vi "RX1.vi"() -> ()   [LabVIEW 2025]
uses:
  <vilib>/addons/Modulation/Analog/support/mod_Set Error Source.vi
  <vilib>/addons/Modulation/Digital/General/MT Generate PSK System Parameters(M).vi
  <vilib>/addons/Modulation/Digital/Support/Common/Validators/mod_Generate Filter Coefficients Validate.vi
  <vilib>/addons/Modulation/Digital/General/subVIs/mod_Generate Filter Coefficients.vi
  <instrlib>/niUSRP/niUSRP Fetch Rx Data (CDB Cluster).vi
  <vilib>/addons/Modulation/niDMT.lvlib
  <vilib>/addons/Modulation/niAMT.lvlib
panel:
  in  "filter parameter":dbl=0.5 format="%.2f"
  out "Waveform Graph 3":cluster{"t0":dbl, "dt":dbl, "Y":dbl[]}(graph)
  out "hamada":errorcluster caption="error out"
  out "error out 6":errorcluster
  out "error out 4":errorcluster
  out "error out 3":errorcluster
  out "error out 2":errorcluster
  out "initiate":errorcluster
  out "output bit stream":i8[](array[numeric])
  out "Waveform Graph 2":cluster{"t0":dbl, "dt":dbl, "Y":dbl[]}(graph)
  out "measurements":T1 {"phase offset (deg)" format="%.2f"; "frequency drift (Hz)" format="%.2f"; "frequency offset (Hz)" format="%.2f"}
  out "IQ Graph":cluster{dbl[], dbl[]} {"?" format="%.2f"; "?" format="%.2f"}
  out "final error out":errorcluster
  in  "active antenna":string="RX2"
  in  "stop":bool
  in  "filter length (symbols)":i32=8
  in  "error in (no error)":errorcluster
  in  "matched samples per symbol (16)":i32=16
  in  "pulse shaping samples per symbol (16)":i32=16
  in  "differential PSK":enum16{"disable", "enable"}(ring)
  in  "M-PSK (4)":i32=8
  in  "samples per symbol (16)":i32=16
  in  "number of samples":i64=1000
  in  "gain":dbl format="%#_6f"
  in  "carrier frequency":dbl=2400000000.0 format="%#_6p"
  in  "IQ rate":dbl=200000.0 format="%#_6p"
  in  "device names":refnum<k15>="NI2900"
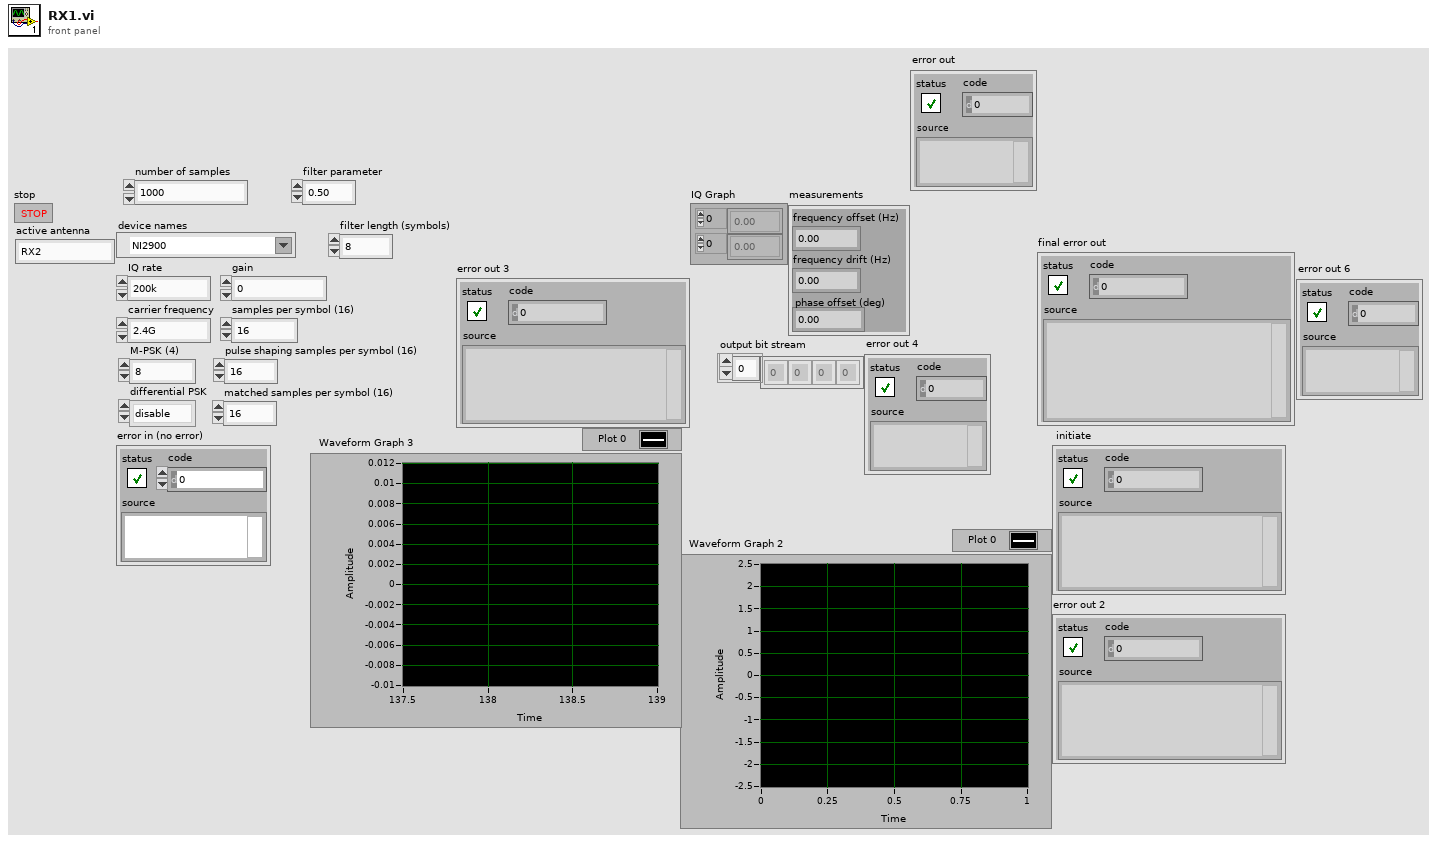
[diagram p1: front panel]
types:
  T1 = cluster{"frequency offset (Hz)":dbl, "frequency drift (Hz)":dbl, "phase offset (deg)":dbl}
  T2 = enum16{"FSK", "PSK", "QAM", "MSK", "PAM", "ASK", "CPM"}
  T3 = enum16{"none", "Raised Cosine", "Root Raised Cos", "Gaussian"}
  T4 = cluster{"samples per symbol (16)":i32, "symbol map":cdb[], "differential PSK":enum16{"disable", "enable"}, "PSK type":u16}
  T5 = typedef "niAMT.lvlib/Complex Data Waveform.ctl" = cluster{"t0":dbl, "dt":dbl, "Y":cdb[]}
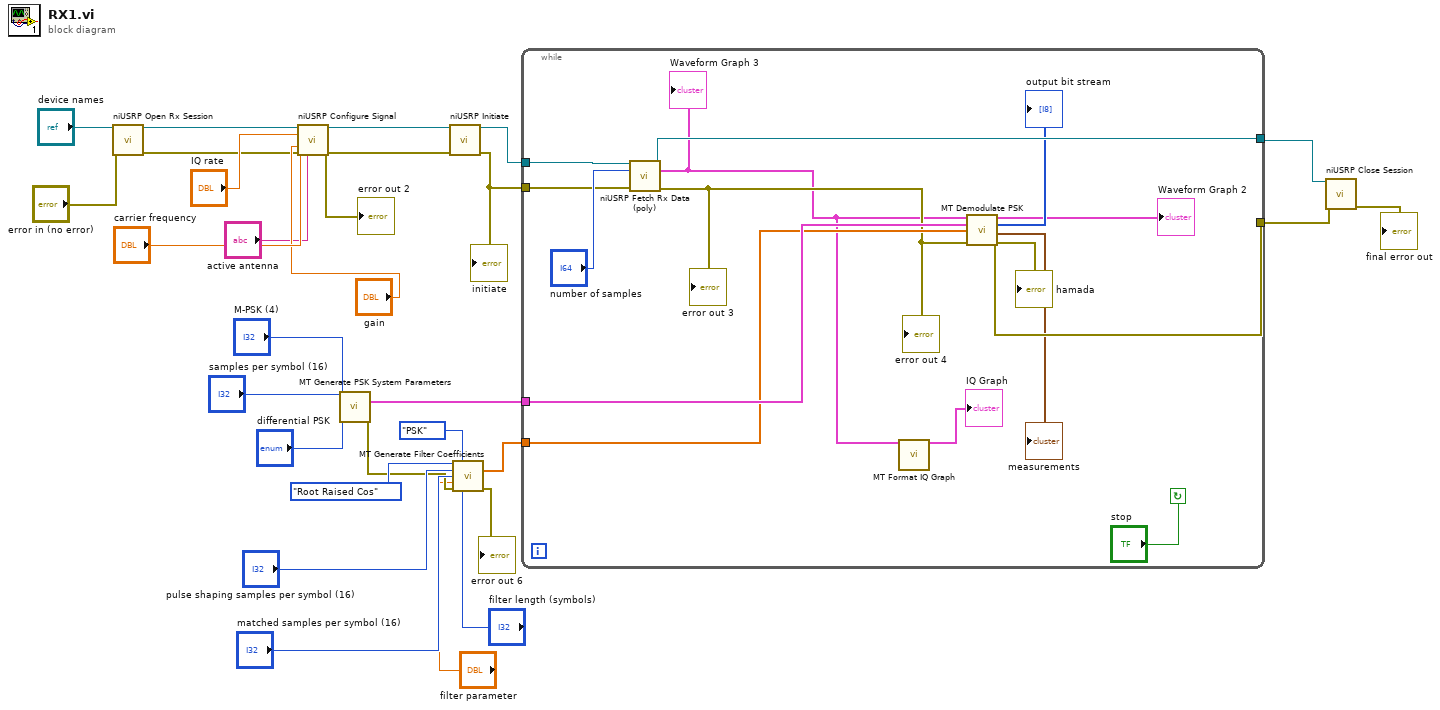
[diagram p0: block diagram]
diagram:
  n1 = call <instrlib>:"niUSRP Open Rx Session.vi"("device names"="device names", "error in (no error)"="error in (no error)") -> ("session handle out"=w27:refnum<k15>, "error out"=w10:errorcluster)  [unwired: 12 in]
  n2 = call <instrlib>:"niUSRP Configure Signal.vi"("session handle"=w27, "IQ rate"="IQ rate", "carrier frequency"="carrier frequency", "gain"="gain", "error in (no error)"=w10, "active antenna"="active antenna") -> ("session handle out"=w23:refnum<k15>, "error out"=w9:errorcluster)  [unwired: 5 in, 3 out]
  "error out 2" <- w9
  n3 = call-poly <vilib>:"MT Generate PSK System Parameters.vi"("samples per symbol (16)"="samples per symbol (16)", "M-PSK (4)"="M-PSK (4)", "differential PSK"="differential PSK") -> ("PSK system parameters"=w17:T4, "error out"=w11:errorcluster)  [unwired: 10 in, 1 out]
  n4 = call <instrlib>:"niUSRP Initiate.vi"("session handle"=w23, "error in (no error)"=w9) -> ("session handle out"=w22:refnum<k15>, "error out"=w8:errorcluster)  [unwired: 12 in]
  "initiate" <- w8
  n5 = call <vilib>:"MT Generate Filter Coefficients.vi"("pulse shaping filter (none)"=T3."Root Raised Cos", "modulation type"=T2."PSK", "pulse shaping samples per symbol (16)"="pulse shaping samples per symbol (16)", "matched samples per symbol (16)"="matched samples per symbol (16)", "filter parameter"="filter parameter", "error in (no error)"=w11, "filter length (symbols)"="filter length (symbols)") -> ("matched filter coefficients"=w16:dbl[], "error out"=→"error out 6":errorcluster)  [unwired: 6 in, 1 out]
  n6 = while {
    tunnel: w22 -> [w42]
    tunnel: [w41] -> w21
    tunnel: w17 -> [w39]
    tunnel: w16 -> [w38]
    tunnel: w8 -> [w37]
    tunnel: [w35] -> w3
    stop <- "stop" continue-if-true
    n7 = call-poly <instrlib>:"niUSRP Fetch Rx Data (poly).vi"("session handle"=w42, "number of samples"="number of samples", "error in (no error)"=w37) -> ("session handle out"=w41:refnum<k15>, "data"=w29:cluster{"t0":dbl, "dt":dbl, "Y":cdb[]}, "error out"=w30:errorcluster)  [unwired: 9 in, 1 out]
    "error out 3" <- w30
    "error out 4" <- w30
    "Waveform Graph 3" <- w29
    n8 = call <vilib>:"MT Format IQ Graph.vi"("IQ data (complex) in"=w29) -> ("IQ Graph"=→"IQ Graph":cluster{dbl[], dbl[]})  [unwired: 13 in, 1 out]
    n9 = call <vilib>:"MT Demodulate PSK.vi"("input complex waveform"=w29, "PSK system parameters"=w39, "matched filter coefficients"=w38, "error in (no error)"=w30) -> ("recovered complex waveform"=→"Waveform Graph 2":T5, "output bit stream"=→"output bit stream":i8[], "measurements"=→"measurements":T1, "error out"=w35:errorcluster)  [unwired: 7 in, 1 out]
    "hamada" <- w35
  }
  n10 = call <instrlib>:"niUSRP Close Session.vi"("session handle"=w21, "error in (no error)"=w3) -> ("error out"=→"final error out":errorcluster)  [unwired: 13 in]
